vi "Transport.vi"(4 "Async Elements":refnum<class "Async Elements.lvclass">, 6 "VI Ref":refnum<vi>, 7 "Actor in":refnum<class "Actor.lvclass">, 10 "Refs":refnum<class "Refs.lvclass">) -> (0 "Error out":errorcluster, 5 "Actor out":refnum<class "Actor.lvclass">)   [LabVIEW 2020, in "jettl.lvlib" / "Event Transport.lvlib"]
uses:
  Event Transport.lvlib
  Actor/Actor.lvclass
  Refs/Refs.lvclass
  Async Elements/Async Elements.lvclass
  Base Async Elements/Base Async Elements/Base Async Elements.lvclass/Base Async Elements.ctl
  Base Attributes/Base Attributes/Base Attributes.lvclass/Base Attributes.ctl
  Event Transport/Event Transport.lvclass/Event Transport.ctl
  Read Msg Ref.vi
  Update Attributes A.vi
  Update Attributes B.vi
  Base Async Elements/Read Async Elements.vi
  Event Transport/Read Msg Ref.vi
  Base Attributes/Init Attributes.vi
  Base Async Elements/Base Async Elements/Read Async Elements.vi
  Base Attributes/Base Attributes/Init Attributes.vi
  Event Transport/Event Transport.lvclass
  C:/git/jettl/src/jettl/jettl/Transport/Transport.lvclass
  Base Attributes/Base Attributes/Base Attributes.lvclass
  C:/git/jettl/src/jettl/jettl/Attributes/Attributes.lvclass
  Call.vi
  Stop jettl Msg/Stop/Stop.vi
  Stop jettl Msg/Stop/Call.vi
  Attributes/Attributes.lvclass
  Base Async Elements/Base Async Elements/Base Async Elements.lvclass
  Msg/Msg.lvclass
  Transport/Transport.lvclass
  jettl.lvlib
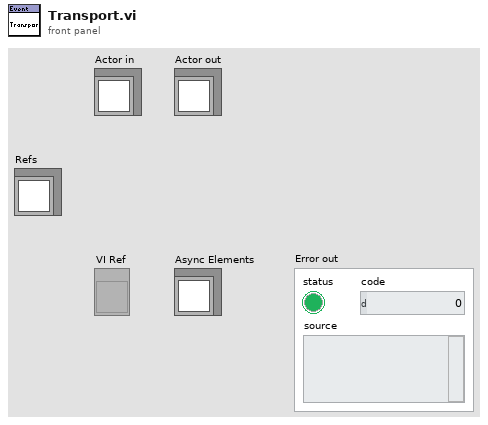
[diagram p1: front panel]
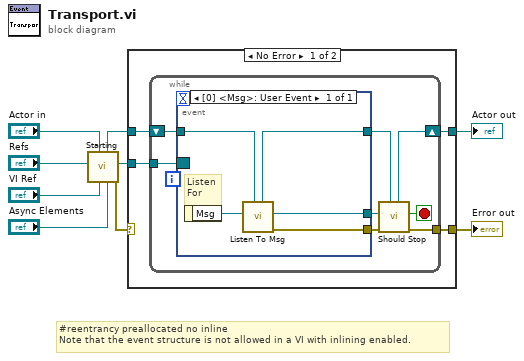
[diagram p0: block diagram]
diagram:
  # "#reentrancy preallocated no inline\nNote that the event structure is not allowed in a VI with inlining enabled."
  n1 = call "Starting.vi"("Async Elements"="Async Elements", "VI Ref"="VI Ref", "Actor in"="Actor in", "Refs"="Refs") -> ("Error out"=w7:errorcluster, "Msg Ref"=w2:refnum<event-registration>, "Actor out"=w8:refnum<class "Actor.lvclass">)  [unwired: 5 in]
  n2 = case shown="No Error" w7 {
    selector: w7 -> [_ w27]
    tunnel: [w10 w28] -> w5
    tunnel: w8 -> [w12 w28]
    tunnel: [w13 w27] -> w9
    tunnel: w2 -> [w11 _]
    frame No Error {
      n3 = while {
        shift-right: [w16] -> w10
        shift-left: w12 -> [w21]
        tunnel: [w19] -> w13
        tunnel: w11 -> [w14]
        stop <- w18 stop-if-true
        n4 = event shown="[0] <Msg>: User Event" {
          selector: w14 -> [_]
          dyn-events: _ -> [_]
          timeout: _ -> [_]
          tunnel: w21 -> [w26]
          tunnel: [w24] -> w15
          tunnel: [w23] -> w20
          tunnel: [w22] -> w17
          event User Event {
            # "Listen\nFor"
            n5 = event-data() -> ("Msg"=w25:refnum<class "Msg.lvclass">)  [unwired: 1 in]
            n6 = call "Listen To Msg.vi"("Actor in"=w26, "Msg"=w25) -> ("Error out"=w23:errorcluster, "Msg Output"=w22:refnum<class "Msg Output.lvclass">, "Actor out"=w24:refnum<class "Actor.lvclass">)  [unwired: 7 in]
          }
        }
        n7 = call "Should Stop.vi"("Actor in"=w15, "Error in"=w20, "Msg Output"=w17) -> ("Error out"=w19:errorcluster, "Stop"=w18:bool, "Actor out"=w16:refnum<class "Actor.lvclass">)  [unwired: 6 in]
      }
    }
    frame Error {
    }
  }
  "Error out" <- w9
  "Actor out" <- w5
